vi "Spike Start Errors.vi"() -> ()   [LabVIEW 2020]
doc: "Manual check of RemoteVI Start.vi's error reporting. Publishes this VI on port with RemoteVI Start.vi, keeps running for hold ms and returns Start's error out and URL; the server ends by itself once this VI is idle. Expected: no error on a free port with no RemoteVI server running in this LabVIEW instance; 5001 while another RemoteVI server runs here (e.g. the fixture on 8089); 60 (from TCP Create Listener in RemoteVI Server Loop.vi) when another process holds the port."
uses:
  source/RemoteVI.lvlib
panel:
  out "error out":errorcluster
  out "URL":string
  in  "hold ms":i32
  in  "port":u16=8090
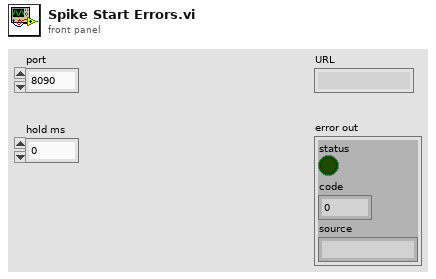
[diagram p1: front panel]
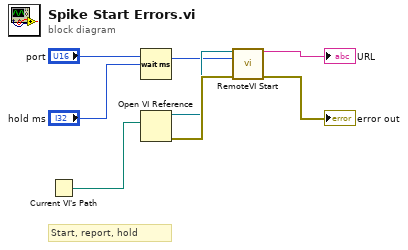
[diagram p0: block diagram]
diagram:
  # "Start, report, hold"
  n1 = Current VI's Path() -> (path=w3:path)
  n2 = Wait (ms)(milliseconds to wait="hold ms") -> ()  [unwired: 1 out]
  n3 = Open VI Reference(vi path=w3) -> (vi reference=w4:refnum<vi>, error out=w5:errorcluster)  [unwired: 5 in]
  n4 = call "RemoteVI Start.vi"("VI"=w4, "port"="port", "error in"=w5) -> ("URL"=→"URL":string, "error out"=→"error out":errorcluster)  [unwired: 11 in]
